vi "thermal_optical_capture_10.vi"() -> ()   [LabVIEW 2025]
panel:
  out "Thermal Preview":T1(plugin-control)
  in  "Stop Preview":bool
  out "Times between Frames":u32
  in  "STOP ACQUISITION":bool
  out "Optical Frame Out":string
  out "Optical Preview":T1(plugin-control)
  in  "Focus":dbl(slide) scale=0.0..100.0
  out "Thermal Frame Out":string
  in  "Output Folder":path
  in  "thermal capture interval (s)":dbl
  in  "Flag Button":bool
  in  "Stop & Save":bool
  in  "Record":bool
  # "Thermal Record"
  # "(Enter \"28\")"
  # "^ append to base data folder \"...\\test_n\\raw\" for nth recording"
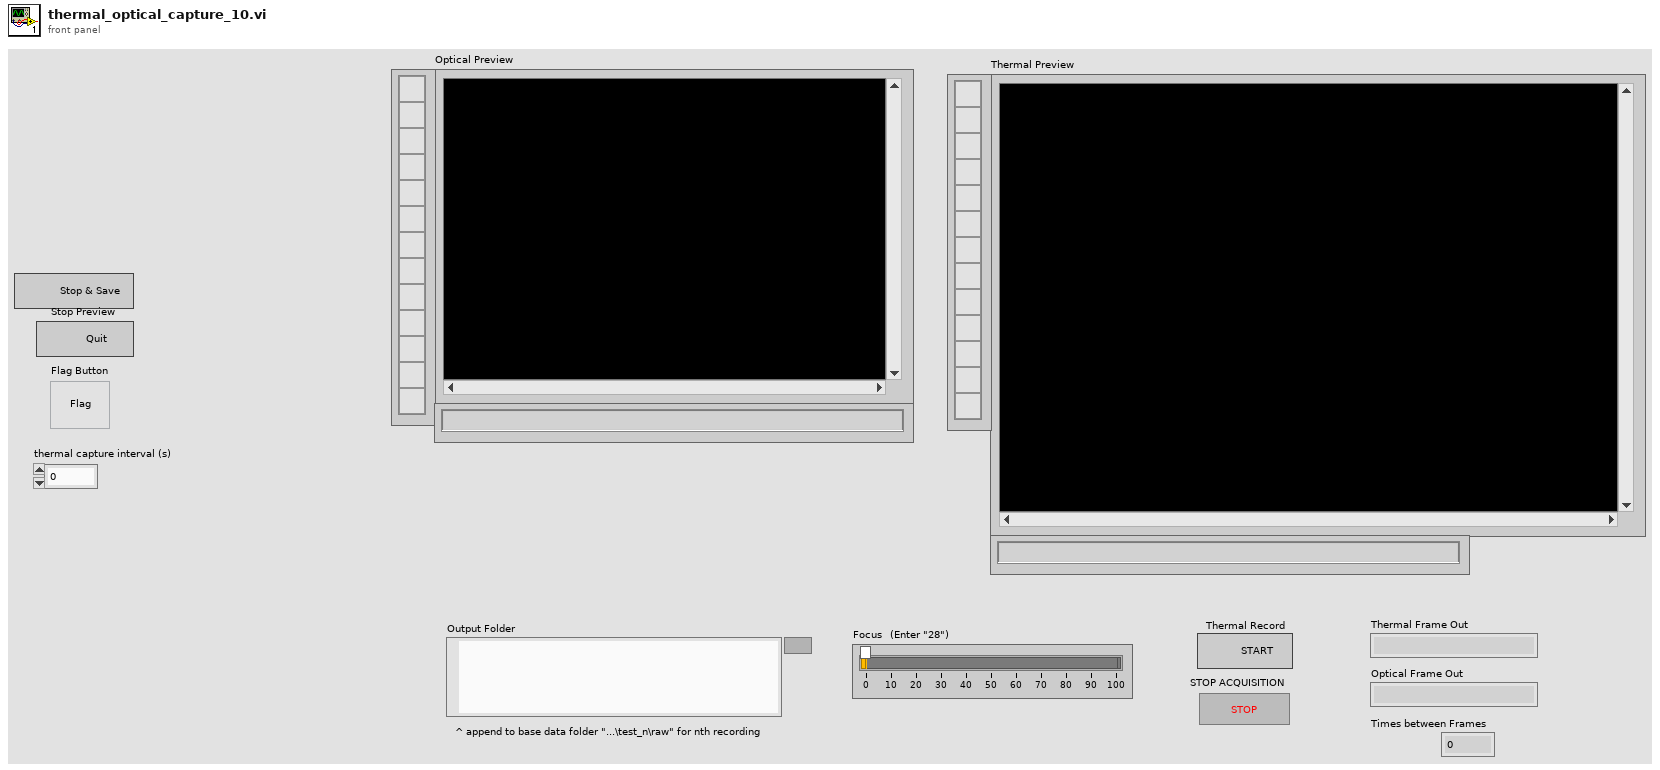
[diagram p1: front panel]
types:
  T1 = typedef "IMAQ Image.ctl" = refnum<image>
  T2 = enum16{"open", "replace", "create", "open or create", "replace or create", "replace or create with confirmation"}
  T3 = enum16{"big-endian, network order", "native, host order", "little-endian"}
  T4 = typedef "Image Type" = u32
  T5 = enum16{"Standard", "Buffered", "CRLF", "Immediate"}
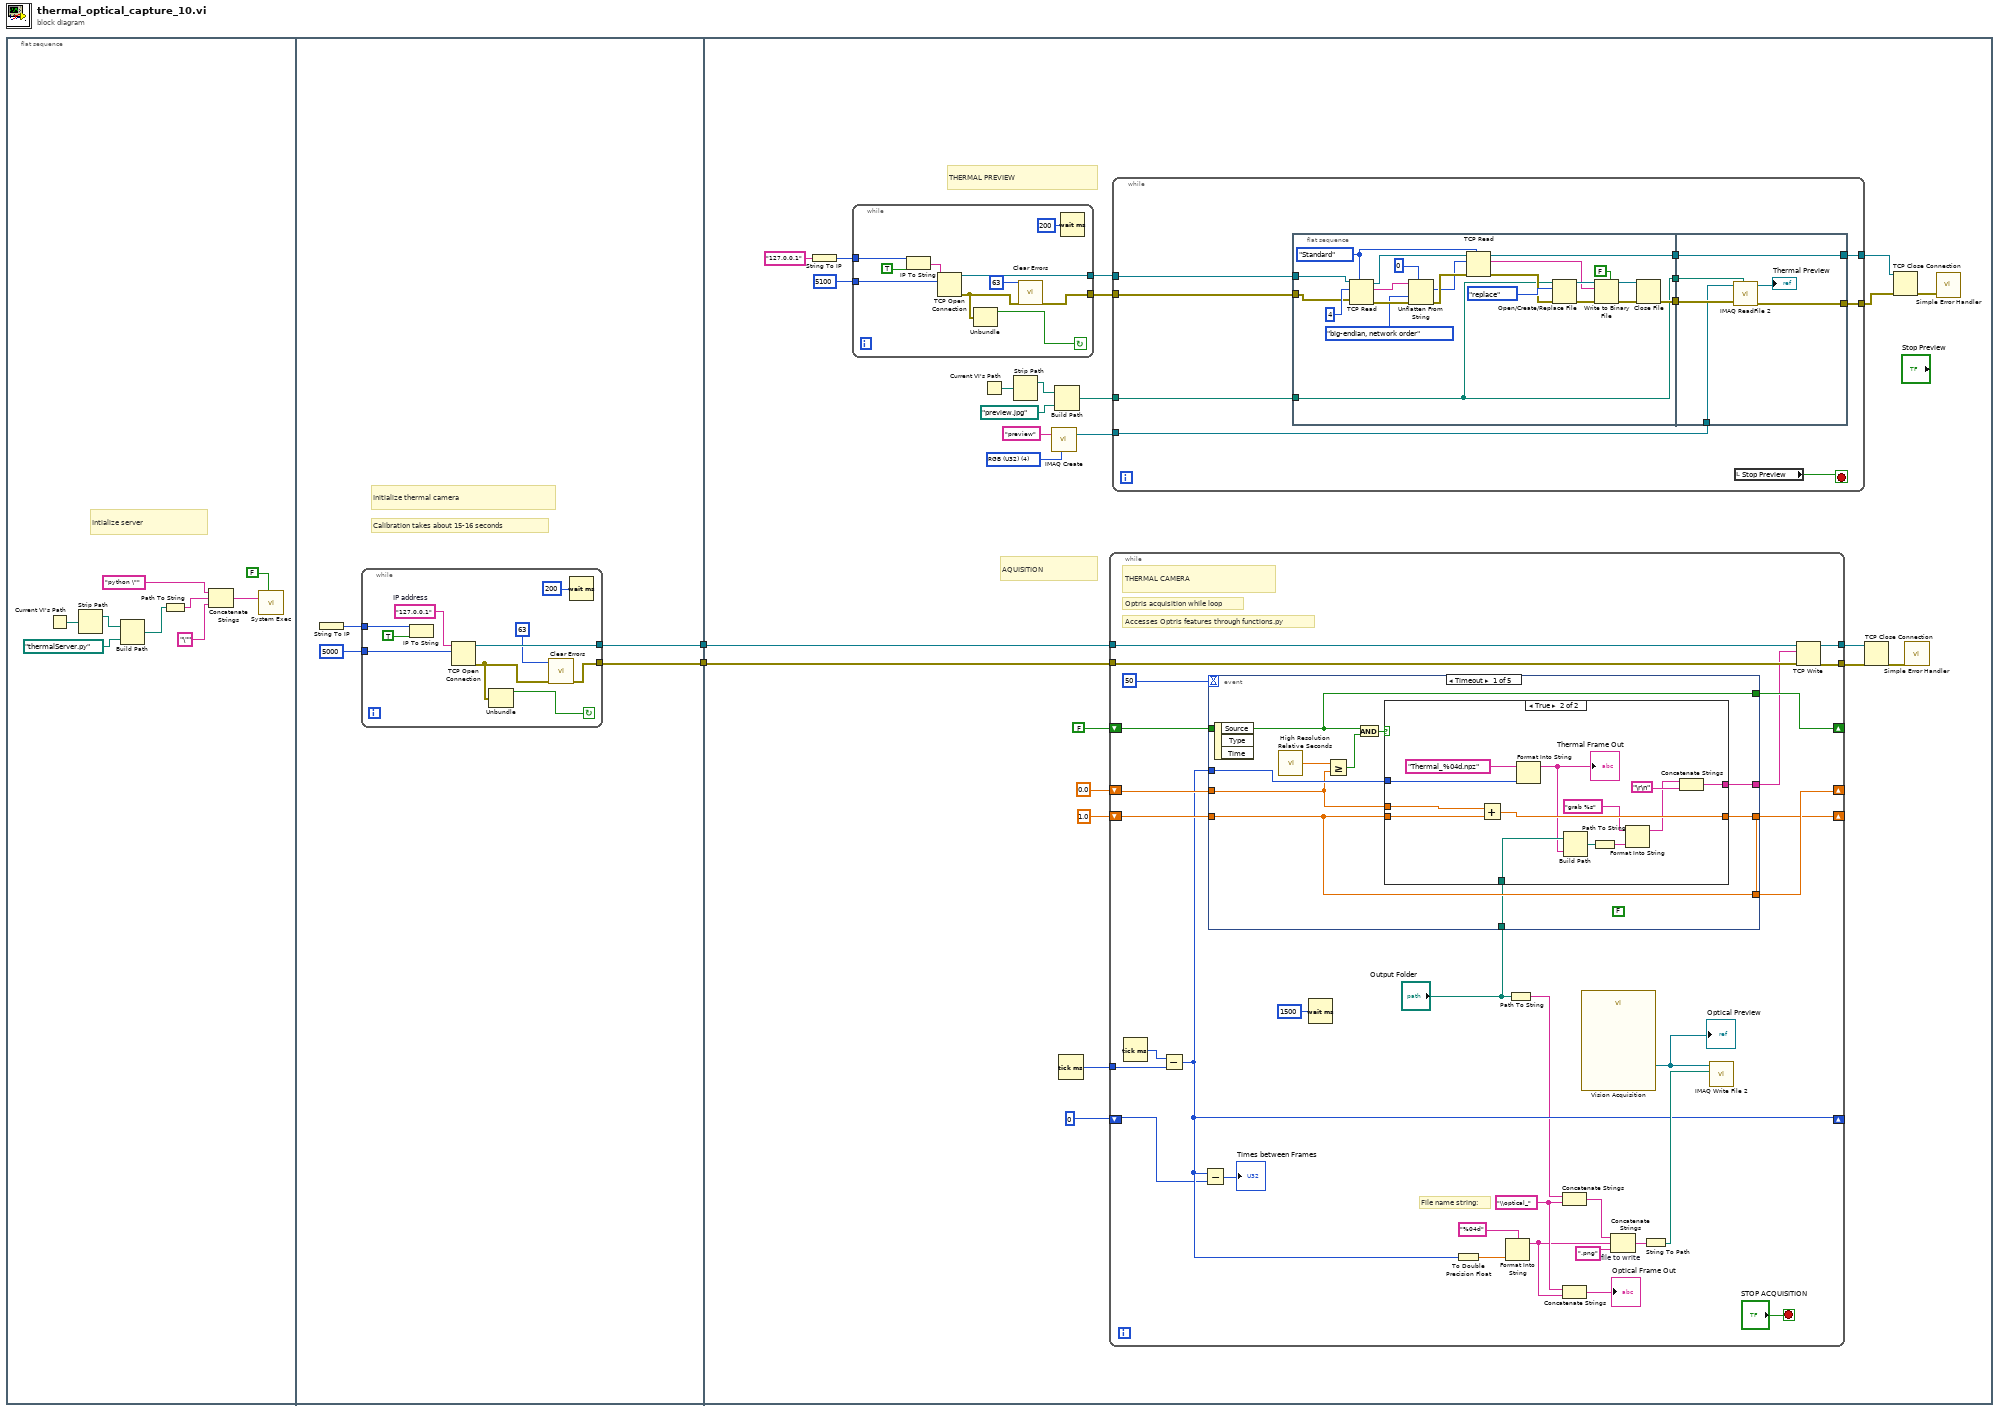
[diagram p0: block diagram]
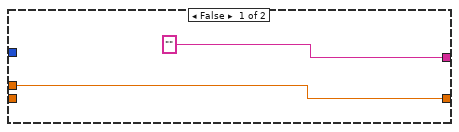
[diagram p2: hidden frame]
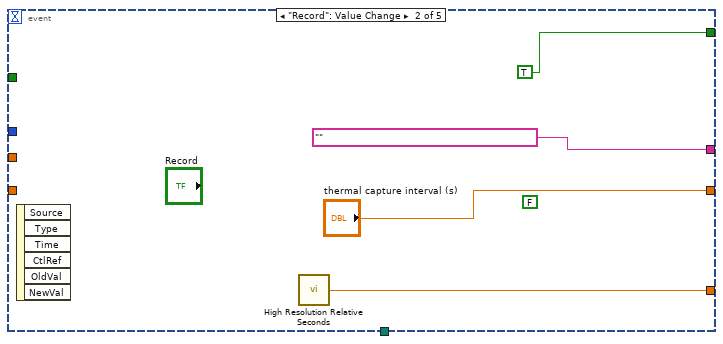
[diagram p3: hidden frame]
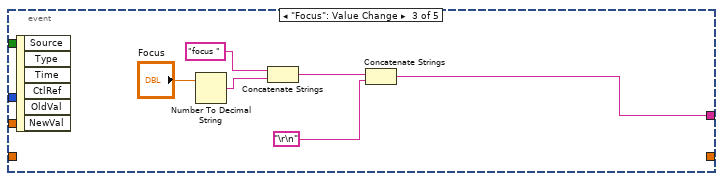
[diagram p4: hidden frame]
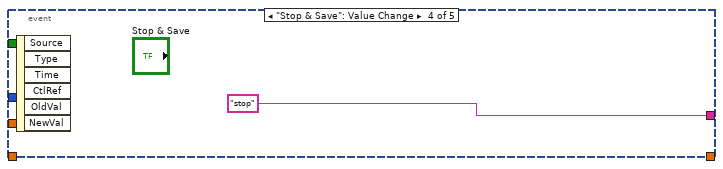
[diagram p5: hidden frame]
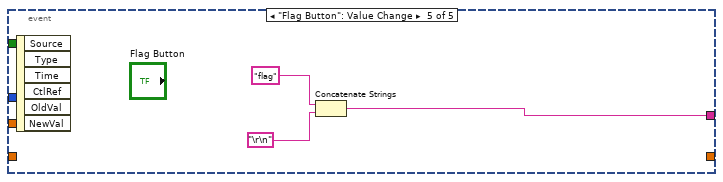
[diagram p6: hidden frame]
diagram:
  n1 = flat-sequence {
    tunnel: [w13] -> w2
    tunnel: [w12] -> w1
    tunnel: w1 -> [w47]
    tunnel: w2 -> [w46]
    frame #0 {
      # "Intialize server"
      n2 = Current VI's Path() -> (path=w6:path)
      n3 = Strip Path(path=w6) -> (stripped path=w7:path)  [unwired: 1 out]
      n4 = Build Path(base path=w7, name or relative path=path "thermalServer.py") -> (appended path=w4:path)
      n5 = Path To String(path=w4) -> (string=w10:string)
      n6 = Concatenate Strings("python \"" ("string"), w10, "\"" ("string")) -> (w9:string)
      n7 = call <vilib>:"System Exec.vi"("wait until completion? (T)"=FALSE, "command line"=w9) -> ()  [unwired: 6 in, 4 out]
    }
    frame #1 {
      # "Initialize thermal camera"
      # "Calibration takes about 15-16 seconds"
      n8 = String To IP() -> (0:w15:u32)  [unwired: 1 in]
      n9 = while {
        tunnel: [w20] -> w13
        tunnel: [w25] -> w12
        tunnel: w15 -> [w24]
        tunnel: u16 5000 ("remote port or service name") -> [w22]
        stop <- w17 continue-if-true
        w16 = "127.0.0.1"  # IP address
        n10 = IP To String(1:TRUE ("dot notation? (F)"), 2:w24) -> ()  [unwired: 1 out]
        n11 = TCP Open Connection(address=w16, remote port or service name=w22) -> (connection ID=w25:refnum<k5>, error out=w21:errorcluster)  [unwired: 3 in]
        n12 = Unbundle(w21) -> ("status"=w17:bool)  [unwired: 2 out]
        n13 = call <vilib>:"Clear Errors.vi"("error in (no error)"=w21, "specific error code to clear (0: all)"=63) -> ("error out"=w20:errorcluster)  [unwired: 4 in, 1 out]
        n14 = Wait (ms)(milliseconds to wait=u32 200) -> ()  [unwired: 1 out]
      }
    }
    frame #2 {
      w31 = T4 4 items=["Grayscale (U8)", "Grayscale (I16)", "Grayscale (SGL)", "Complex (CSG)", "RGB (U32)", "HSL (U32)", "RGB (U64)", "Grayscale (U16)"] ("Image Type")
      # "THERMAL PREVIEW"
      # "AQUISITION"
      n15 = String To IP(1:"127.0.0.1" ("name")) -> (0:w30:u32)
      n16 = while {
        tunnel: w30 -> [w60]
        tunnel: [w54] -> w29
        tunnel: [w58] -> w28
        tunnel: u16 5100 ("remote port or service name") -> [w56]
        stop <- w51 continue-if-true
        n17 = IP To String(1:TRUE ("dot notation? (F)"), 2:w60) -> (0:w59:string)
        n18 = TCP Open Connection(address=w59, remote port or service name=w56) -> (connection ID=w58:refnum<k5>, error out=w55:errorcluster)  [unwired: 3 in]
        n19 = Unbundle(w55) -> ("status"=w51:bool)  [unwired: 2 out]
        n20 = call <vilib>:"Clear Errors.vi"("error in (no error)"=w55, "specific error code to clear (0: all)"=63) -> ("error out"=w54:errorcluster)  [unwired: 4 in, 1 out]
        n21 = Wait (ms)(milliseconds to wait=u32 200) -> ()  [unwired: 1 out]
      }
      n22 = Current VI's Path() -> (path=w39:path)
      n23 = Strip Path(path=w39) -> (stripped path=w40:path)  [unwired: 1 out]
      n24 = call "IMAQ Create"("Image Name"="preview", "Image Type"=w31) -> ("New Image"=w35:T1)  [unwired: 3 in, 1 out]
      n25 = Build Path(base path=w40, name or relative path=path "preview.jpg") -> (appended path=w38:path)
      n26 = Tick Count (ms)() -> (millisecond timer value=w42:u32)
      n27 = while {
        tunnel: [w129] -> w48
        tunnel: [w128] -> w49
        tunnel: w47 -> [w127]
        tunnel: w46 -> [w126]
        shift-right: [w125] -> _
        shift-left: 0.0 -> [w121]
        shift-right: [w122] -> _
        shift-left: 1.0 -> [w119]
        shift-right: [w123] -> _
        shift-left: FALSE -> [w120]
        tunnel: w42 -> [w104]
        shift-right: [w103] -> _
        shift-left: u32 0 -> [w102]
        stop <- "STOP ACQUISITION" stop-if-true
        w113 = "\\optical_" ("string")
        # "File name string:"
        # "THERMAL CAMERA"
        # "Optris acquisition while loop"
        # "Accesses Optris features through functions.py"
        n28 = Tick Count (ms)() -> (millisecond timer value=w105:u32)
        n29 = Subtract(x=w105, y=w104) -> (x-y=w103:u32)
        n30 = Subtract(x=w103, y=w102) -> (x-y=→"Times between Frames":u32)
        n31 = event shown="[0] Timeout" {
          selector: _ -> [_ _ _ _ _]
          dyn-events: _ -> [_ _ _ _ _]
          timeout: 50 -> [_ _ _ _ _]
          tunnel: [w135 "" w159 "stop" w168] -> w118
          tunnel: w103 -> [w136 _ _ _ _]
          tunnel: [w133 w158 _ _ _] -> w125
          tunnel: [w131 TRUE _ _ _] -> w123
          tunnel: [w132 "thermal capture interval (s)" _ _ _] -> w122
          tunnel: w121 -> [w134 _ _ _ _]
          tunnel: w120 -> [w131 _ _ _ _]
          tunnel: w119 -> [w132 _ _ _ _]
          tunnel: "Output Folder" -> [w130 _ _ _ _]
          event Timeout {
            (unwired) FALSE
            n32 = event-data() -> ()  [unwired: 1 in, 3 out]
            n33 = call <vilib>:"High Resolution Relative Seconds.vi"() -> ("relative seconds"=w139:dbl)
            n34 = Greater Or Equal?(x=w139, y=w134) -> (x >= y?=w138:bool)
            n35 = And(x=w131, y=w138) -> (x .and. y?=w137:bool)
            n36 = case shown="True" w137 {
              tunnel: w136 -> [_ w152]
              tunnel: ["" w153] -> w135
              tunnel: w134 -> [w140 w151]
              tunnel: w132 -> [_ w150]
              tunnel: [w140 w149] -> w133
              tunnel: w130 -> [_ w143]
              frame False {
              }
              frame True {
                n37 = Add(x=w151, y=w150) -> (x+y=w149:dbl)
                n38 = Format Into String(format string="Thermal_%04d.npz", w152) -> (resulting string=w142:string)  [unwired: 2 in, 1 out]
                "Thermal Frame Out" <- w142
                n39 = Build Path(base path=w143, name or relative path=w142) -> (appended path=w147:path)
                n40 = Path To String(path=w147) -> (string=w145:string)
                n41 = Format Into String(format string="grab %s", w145) -> (resulting string=w144:string)  [unwired: 2 in, 1 out]
                n42 = Concatenate Strings(w144, "\r\n") -> (w153:string)
              }
            }
          }
          event "Record": Value Change {
            (unwired) FALSE
            n43 = event-data() -> ()  [unwired: 1 in, 6 out]
            n44 = call <vilib>:"High Resolution Relative Seconds.vi"() -> ("relative seconds"=w158:dbl)
          }
          event "Focus": Value Change {
            n45 = event-data() -> ()  [unwired: 1 in, 6 out]
            n46 = Number To Decimal String(number="Focus") -> (decimal integer string=w164:string)  [unwired: 1 in]
            n47 = Concatenate Strings("focus ", w164) -> (w161:string)
            n48 = Concatenate Strings(w161, "\r\n") -> (w159:string)
          }
          event "Stop & Save": Value Change {
            n49 = event-data() -> ()  [unwired: 1 in, 6 out]
          }
          event "Flag Button": Value Change {
            n50 = event-data() -> ()  [unwired: 1 in, 6 out]
            n51 = Concatenate Strings("flag", "\r\n") -> (w168:string)
          }
        }
        n52 = Wait (ms)(milliseconds to wait=u32 1500) -> ()  [unwired: 1 out]
        n53 = To Double Precision Float(number=w103) -> (double precision float=w111:dbl)
        n54 = Format Into String(format string="%04d" ("time format string (%c)"), w111) -> (resulting string=w109:string)  [unwired: 2 in, 1 out]
        n55 = Path To String(path="Output Folder") -> (string=w99:string)
        n56 = Concatenate Strings(w99, w113) -> (w114:string)
        n57 = Concatenate Strings(w113, w109) -> (→"Optical Frame Out":string)
        n58 = call "Vision Acquisition"() -> ("Image Out"=w117:T1)  [unwired: 26 in, 1 out]
        "Optical Preview" <- w117
        n59 = Concatenate Strings "file to write"(w114, w109, ".png" ("string")) -> (w116:string)
        n60 = String To Path(string=w116) -> (path=w110:path)
        n61 = call-poly "IMAQ Write File 2"("File Path"=w110, "Image"=w117) -> ()  [unwired: 8 in, 2 out]
        n62 = TCP Write(connection ID=w127, data in=w118, error in (no error)=w126) -> (connection ID out=w128:refnum<k5>, error out=w129:errorcluster)  [unwired: 1 in, 1 out]
      }
      n63 = while {
        tunnel: w35 -> [w65]
        tunnel: [w66] -> w36
        tunnel: [w70] -> w37
        tunnel: w38 -> [w68]
        tunnel: w29 -> [w63]
        tunnel: w28 -> [w62]
        stop <- w61 stop-if-true
        n64 = flat-sequence {
          tunnel: w68 -> [w74]
          tunnel: [w76] -> w69
          tunnel: [w75] -> w67
          tunnel: [w74] -> w64
          tunnel: w63 -> [w72]
          tunnel: w62 -> [w71]
          tunnel: [w98] -> w70
          tunnel: w69 -> [w98]
          tunnel: w67 -> [w97]
          tunnel: [w96] -> w66
          tunnel: w65 -> [w95]
          tunnel: w64 -> [w94]
          frame #0 {
            w85 = T5."Standard" ("mode (standard)")
            n65 = TCP Read(connection ID=w71, bytes to read=4, error in (no error)=w72, 7:w85) -> (connection ID out=w88:refnum<k5>, data out=w73:string, error out=w91:errorcluster)  [unwired: 1 in]
            n66 = Unflatten From String(type=0, binary string=w73, byte order (0:big-endian, network order)=T3."big-endian, network order", error in (no error)=w91) -> (value=w86:i32, error out=w87:errorcluster)  [unwired: 1 in, 1 out]
            n67 = TCP Read(connection ID=w88, bytes to read=w86, error in (no error)=w87, 7:w85) -> (connection ID out=w76:refnum<k5>, data out=w81:string, error out=w83:errorcluster)  [unwired: 1 in]
            n68 = Open/Create/Replace File(file path (use dialog)=w74, error in=w83, operation (0:open)=T2."replace") -> (refnum out=w82:refnum<file>, error out=w79:errorcluster)  [unwired: 3 in, 1 out]
            n69 = Write to Binary File(file (use dialog)=w82, data=w81, error in=w79, 5:FALSE ("prepend array or string size? (T)")) -> (refnum out=w77:refnum<file>, error out=w78:errorcluster)  [unwired: 2 in, 1 out]
            n70 = Close File(refnum=w77, error in=w78) -> (error out=w75:errorcluster)  [unwired: 1 out]
          }
          frame #1 {
            n71 = call "IMAQ ReadFile 2"("File Path"=w94, "error in (no error)"=w97, "Image"=w95) -> ("error out"=w96:errorcluster, "Image Out"=→"Thermal Preview":T1)  [unwired: 4 in, 3 out]
          }
        }
        n72 = local read "Stop Preview"() -> (w61:bool)
      }
      n73 = TCP Close Connection(connection ID=w49, error in (no error)=w48) -> (error out=w50:errorcluster)  [unwired: 1 in, 1 out]
      n74 = TCP Close Connection(connection ID=w37, error in (no error)=w36) -> (error out=w34:errorcluster)  [unwired: 1 in, 1 out]
      n75 = call <vilib>:"Simple Error Handler.vi"("error in (no error)"=w50) -> ()  [unwired: 4 in, 5 out]
      n76 = call <vilib>:"Simple Error Handler.vi"("error in (no error)"=w34) -> ()  [unwired: 4 in, 5 out]
    }
  }
